vi "ACC.vi"(3 "Acc":dbl format="%#_13g", 4 "Max S":dbl format="%#_13g", 5 "Target":dbl format="%#_13g") -> (0 "Speed":dbl[](graph), 1 "Position":dbl[](graph))   [LabVIEW 2019]
panel:
  out "Array 4":dbl[](array[numeric])
  out "sum":dbl
  out "Array 3":dbl[](array[numeric])
  out "Array 2":dbl[](array[numeric])
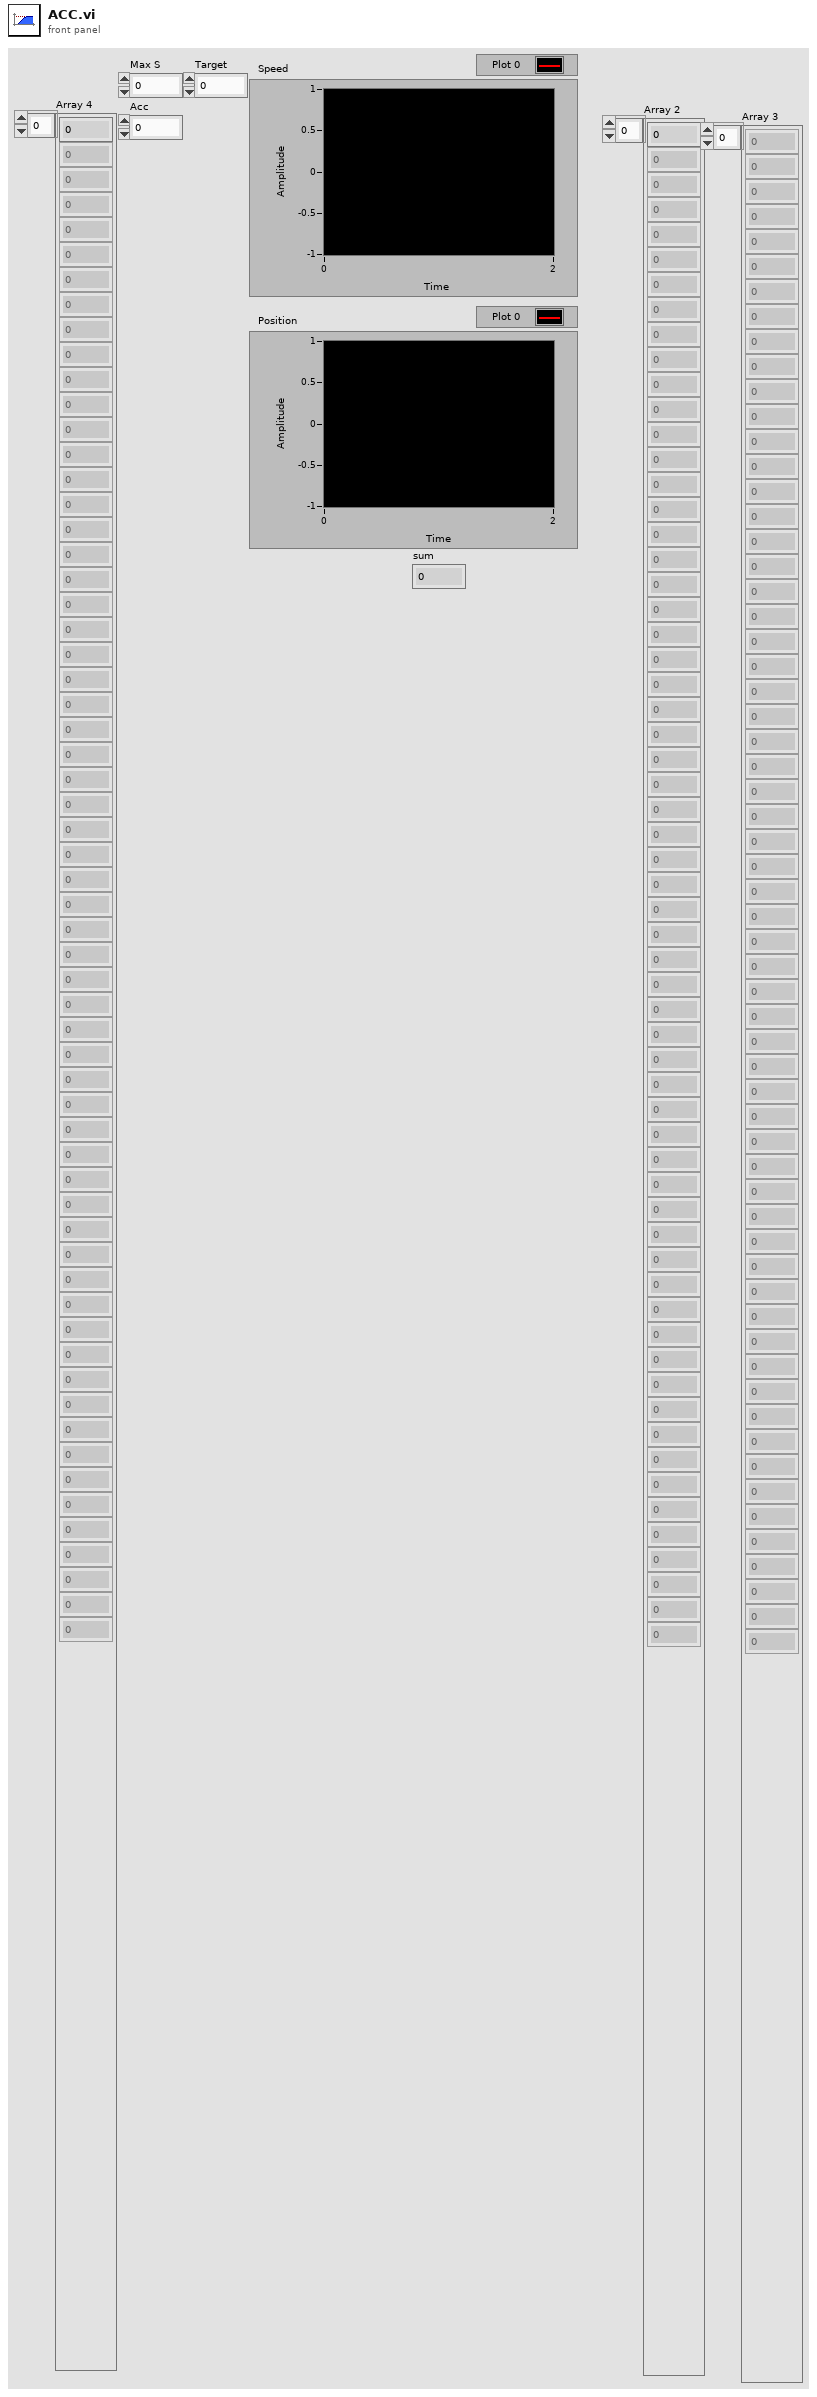
[diagram p1: front panel]
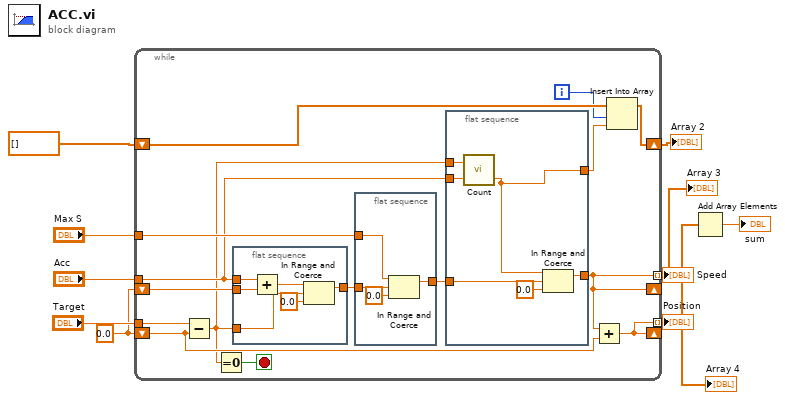
[diagram p0: block diagram]
diagram:
  w1 = 0.0
  n1 = while {
    tunnel: "Max S" -> [w20]
    tunnel: "Acc" -> [w17]
    tunnel: "Target" -> [w23]
    shift-right: [w14] -> _
    shift-left: w1 -> [w24]
    shift-right: [w15] -> _
    shift-left: w1 -> [w22]
    tunnel: [w15] -> w2 mode=indexing
    tunnel: [w14] -> w5 mode=indexing
    shift-right: [w13] -> w3
    shift-left: dbl[] [] ("Array") -> [w12]
    i -> [w10]
    stop <- w19 stop-if-true
    n2 = Subtract(x=w23, y=w22) -> (x-y=w16:dbl)
    n3 = Equal To 0?(x=w16) -> (x = 0?=w19:bool)
    n4 = flat-sequence {
      tunnel: w24 -> [w40]
      tunnel: w17 -> [w39]
      tunnel: w16 -> [w37]
      tunnel: [w35] -> w21
      frame #0 {
        n5 = Add(x=w39, y=w40) -> (x+y=w38:dbl)
        n6 = In Range and Coerce(upper limit=w38, x=w37, lower limit=0.0) -> (coerced(x)=w35:dbl)  [unwired: 1 out]
      }
    }
    n7 = flat-sequence {
      tunnel: w21 -> [w34]
      tunnel: w20 -> [w32]
      tunnel: [w31] -> w18
      frame #0 {
        n8 = In Range and Coerce(upper limit=w32, x=w34, lower limit=0.0) -> (coerced(x)=w31:dbl)  [unwired: 1 out]
      }
    }
    n9 = flat-sequence {
      tunnel: w18 -> [w30]
      tunnel: w17 -> [w28]
      tunnel: w16 -> [w27]
      tunnel: [w26] -> w14
      tunnel: [w25] -> w11
      frame #0 {
        n10 = call "Count.vi"("A"=w28, "S"=w27) -> ("sqrt(x)"=w25:dbl)  [unwired: 1 out]
        n11 = In Range and Coerce(upper limit=w25, x=w30, lower limit=0.0) -> (coerced(x)=w26:dbl)  [unwired: 1 out]
      }
    }
    n12 = Add(x=w14, y=w22) -> (x+y=w15:dbl)
    n13 = Insert Into Array(array=w12, index=w10, new element=w11) -> (w13:dbl[])
  }
  "Position" <- w2
  "Speed" <- w5
  "Array 2" <- w3
  "Array 3" <- w5
  "Array 4" <- w2
  n14 = Add Array Elements(numeric array=w2) -> (sum=→"sum":dbl)
